vi "Log_Write.vi"(4 "Right Count":u16, 5 "Left Count":u16, 6 "error in":errorcluster, 8 "Text":string, 9 "Code":u16, 10 "Event":string, 11 "Log Dir":path) -> (3 "error out":errorcluster)   [LabVIEW 2018]
doc: "Use this template to build a VI to use as a subVI."
panel:
  # "說明：在 logs 資料夾的當天 CSV 後面加一行，新檔先寫標題。\n用 open or create，不能用 replace。"
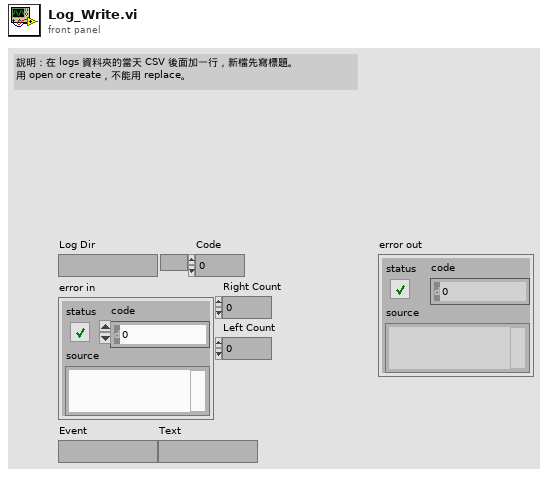
[diagram p1: front panel]
types:
  T1 = enum16{"open", "replace", "create", "open or create", "replace or create", "replace or create with confirmation"}
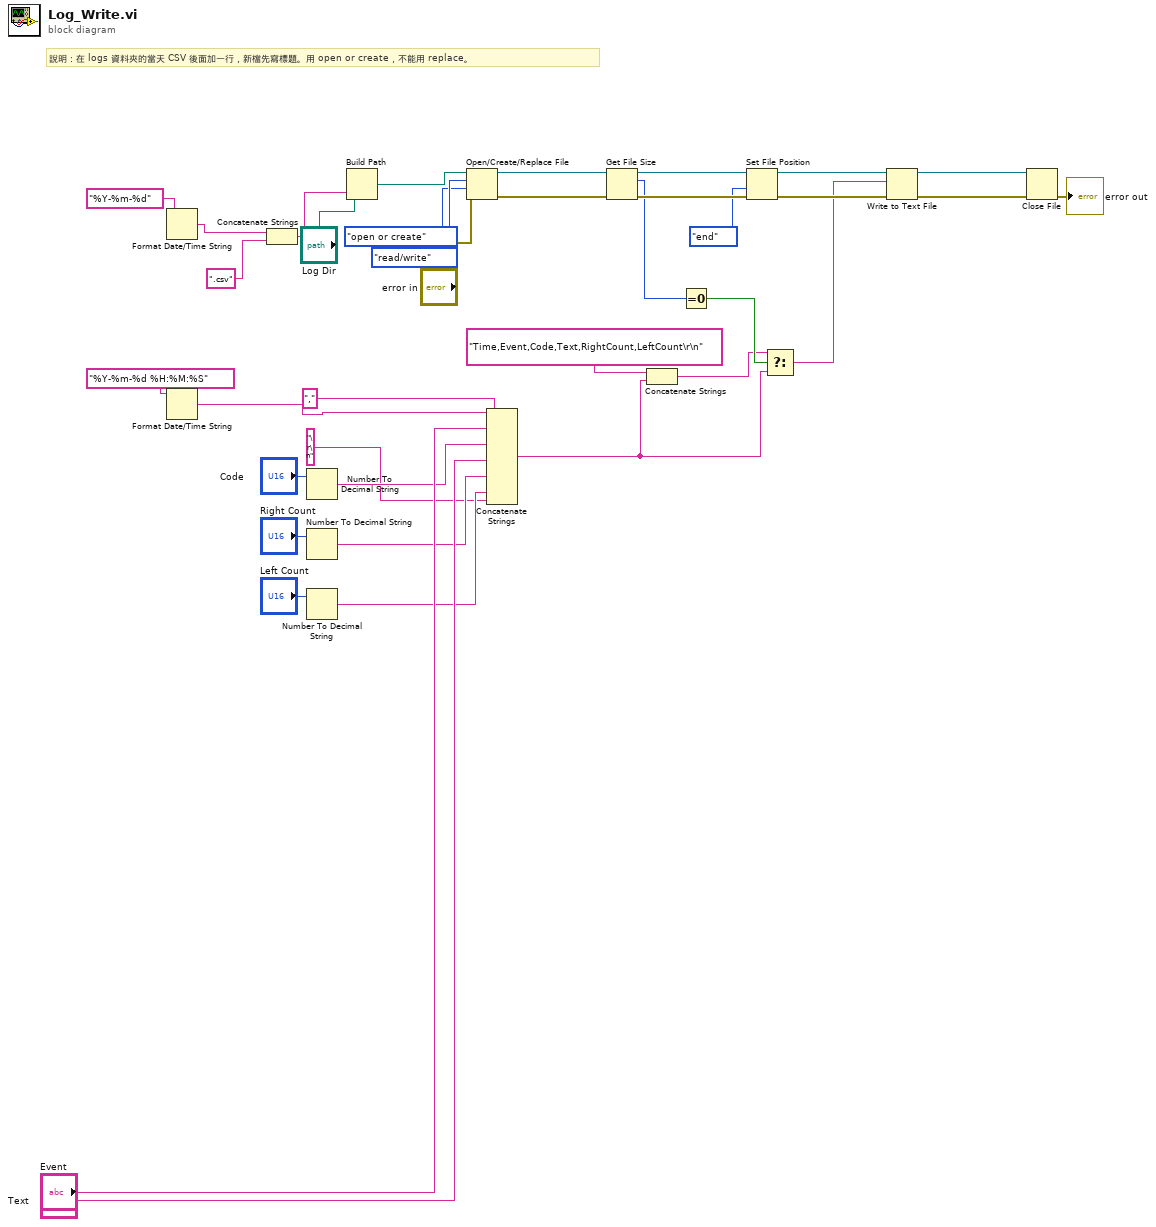
[diagram p0: block diagram]
diagram:
  w18 = ","
  # "說明：在 logs 資料夾的當天 CSV 後面加一行，新檔先寫標題。用 open or create，不能用 replace。"
  n1 = Format Date/Time String(time format string (%c)="%Y-%m-%d") -> (date/time string=w35:string)  [unwired: 2 in]
  n2 = Format Date/Time String(time format string (%c)="%Y-%m-%d %H:%M:%S") -> (date/time string=w19:string)  [unwired: 2 in]
  n3 = Concatenate Strings(w35, ".csv") -> (w33:string)
  n4 = Number To Decimal String(number="Code") -> (decimal integer string=w16:string)  [unwired: 1 in]
  n5 = Number To Decimal String(number="Right Count") -> (decimal integer string=w14:string)  [unwired: 1 in]
  n6 = Number To Decimal String(number="Left Count") -> (decimal integer string=w13:string)  [unwired: 1 in]
  n7 = Build Path(base path="Log Dir", name or relative path=w33) -> (appended path=w32:path)
  n8 = Open/Create/Replace File(file path (use dialog)=w32, error in="error in", operation (0:open)=T1."open or create", access (0:read/write)=enum16{"read/write", "read-only", "write-only"}."read/write") -> (refnum out=w28:refnum<file>, error out=w27:errorcluster)  [unwired: 2 in, 1 out]
  n9 = Concatenate Strings(w19, w18, "Event", w18, w16, w18, "Text", w18, w14, w18, w13, "\r\n") -> (w9:string)
  n10 = Get File Size(file=w28, error in=w27) -> (refnum out=w26:refnum<file>, size (in bytes)=w11:i64, 0:w25:errorcluster)
  n11 = Concatenate Strings("Time,Event,Code,Text,RightCount,LeftCount\r\n", w9) -> (w7:string)
  n12 = Equal To 0?(x=w11) -> (x = 0?=w8:bool)
  n13 = Set File Position(refnum=w26, from (0:start)=enum16{"start", "end", "current"}."end", error in=w25) -> (refnum out=w6:refnum<file>, error out=w5:errorcluster)  [unwired: 1 in]
  n14 = Select(t=w7, s=w8, f=w9) -> (s? t:f=w4:string)
  n15 = Write to Text File(file (use dialog)=w6, text=w4, error in=w5) -> (refnum out=w3:refnum<file>, error out=w2:errorcluster)  [unwired: 1 in, 1 out]
  n16 = Close File(refnum=w3, error in=w2) -> (error out=→"error out":errorcluster)  [unwired: 1 out]
